vi "macro_LinearFilter_ExecuteTC.vi"   [LabVIEW 2019, in "Trajectory_Library.lvlib"]
uses:
  Trajectory_Library.lvlib
  LinearFilter_LP_BW1_Execute.vi
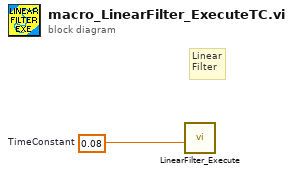
[diagram p0: block diagram]
diagram:
  w1 = 0.08  # TimeConstant
  # "Linear\nFilter"
  n1 = call-poly "LinearFilter_Execute.vi"("TimeConstant"=w1) -> ()  [unwired: 10 in, 1 out]
